vi "SPARK Persist Parameters.vi"(8 "error in":errorcluster, 11 "Spark refnum":T1) -> (0 "error out":errorcluster, 3 "Spark refnum":T1)   [LabVIEW 2023, in "REVLibDriver.lvlib"]
doc: "Save all parameters to the SPARK's non-volatile memory after setting the given configuration. This will allow parameters to persist across power cycles."
uses:
  <vilib>/REVLibDriver/REVLibDriver.lvlib
  <vilib>/REV Custom Controls/REVSparkRefnum.ctl
  REVLibDriver.so
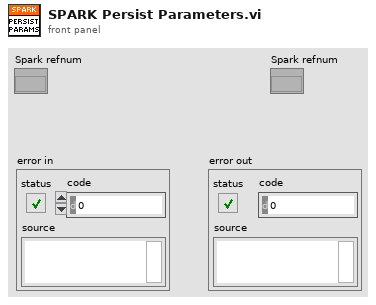
[diagram p1: front panel]
types:
  T1 = typedef "REVLibDriver.lvlib/REVSparkRefnum.ctl" = refnum<k20>
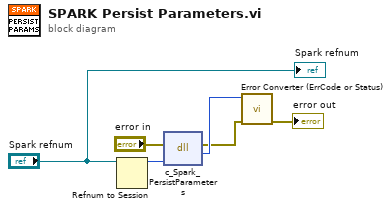
[diagram p0: block diagram]
diagram:
  n1 = Refnum to Session(7:"Spark refnum") -> (3:w1:u64)  [unwired: 1 in, 1 out]
  n2 = dll-call lib="REVLibDriver.*" fn="c_Spark_PersistParameters"(error in="error in", "handle"=w1) -> (error out=w4:errorcluster, "return type"=w5:u32)  [unwired: 3 in, 1 out]
  n3 = call <vilib>:"Error Converter (ErrCode or Status).vi"("error in (no error)"=w4, "error code"=w5) -> ("error out"=→"error out":errorcluster)  [unwired: 9 in]
  "Spark refnum" <- "Spark refnum"
